vi "from string.vi"(8 "error in":errorcluster, 9 "data":string, 10 "version":string, 11 "CVT configuration in":refnum<class "CVT configuration.lvclass">) -> (0 "error out":errorcluster, 3 "CVT configuration out":refnum<class "CVT configuration.lvclass">)   [LabVIEW 2013, in "CVT configuration.lvclass"]
doc: "Provides an interface for loading a module configuration from a file or other serialized data source. It is recommended that all children of this class store data in two sets--data required for its own initialization, and any data required for parent initialization--and that each implementation uses the <b>Call Parent Method</b> primitive to de-serialize parent information. As a result, it is expected that every module configuration class calls <b>component configuration.lvclass:From String.vi</b>."
uses:
  CVT configuration.lvclass
  <vilib>/NI/Tag Bus Module Framework/channel/TBM channel.lvclass
  <vilib>/NI/Tag Bus Module Framework/module configuration/TBM module configuration.lvclass
  CVT configuration.lvclass/CVT configuration.ctl
  <vilib>/NI/Configuration Framework/serializable configuration/NISE_CEF_serializable configuration.lvclass
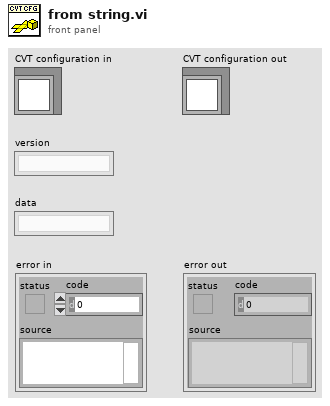
[diagram p1: front panel]
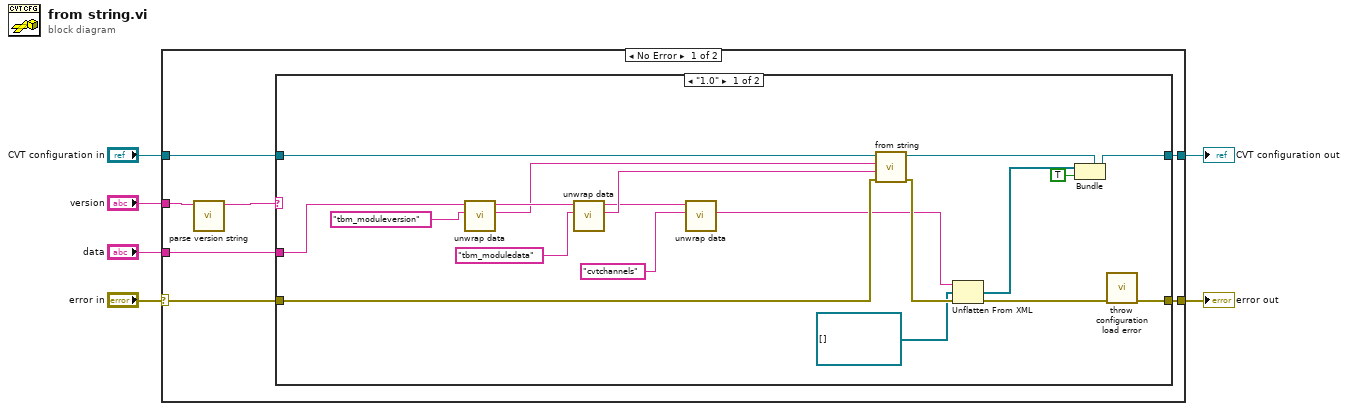
[diagram p0: block diagram]
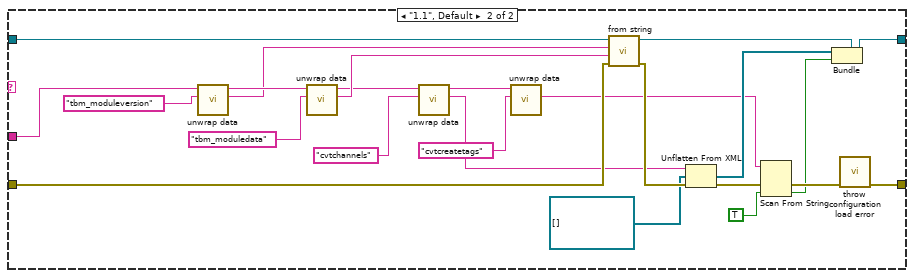
[diagram p2: hidden frame]
diagram:
  n1 = case shown="No Error" "error in" {
    selector: "error in" -> [w7 w58]
    tunnel: "data" -> [w13 _]
    tunnel: "CVT configuration in" -> [w12 w57]
    tunnel: [w11 w57] -> w5
    tunnel: [w10 w58] -> w4
    tunnel: "version" -> [w9 _]
    frame No Error {
      n2 = call <vilib>:"parse version string.vi"("full version"=w9) -> ("major.minor version"=w8:string)  [unwired: 7 in, 3 out]
      n3 = case shown="\"1.0\"" w8 {
        tunnel: w13 -> [w27 w51]
        tunnel: w7 -> [w26 w50]
        tunnel: w12 -> [w32 w56]
        tunnel: [w21 w45] -> w11
        tunnel: [w29 w53] -> w10
        frame "1.0" {
          n4 = call <vilib>:"unwrap data.vi"("identifier"="tbm_moduleversion" ("additional identifier"), "data to unwrap"=w27) -> ("unwrapped data"=w22:string, "remaining string"=w28:string)  [unwired: 8 in]
          n5 = call <vilib>:"unwrap data.vi"("identifier"="tbm_moduledata" ("additional identifier"), "data to unwrap"=w28) -> ("unwrapped data"=w24:string, "remaining string"=w17:string)  [unwired: 8 in]
          n6 = call <vilib>:"unwrap data.vi"("identifier"="cvtchannels" ("additional identifier"), "data to unwrap"=w17) -> ("unwrapped data"=w15:string)  [unwired: 8 in, 1 out]
          n7 = call-parent "from string.vi"("error in"=w26, "data"=w24, "version"=w22, "module configuration in"=w32) -> ("error out"=w30:errorcluster, "module configuration out"=w31:refnum<class "CVT configuration.lvclass">)  [unwired: 6 in]
          n8 = Unflatten From XML(xml string=w15, type=refnum<class "TBM channel.lvclass">[] [] ("channels"), error in (no error)=w30) -> (value=w18:refnum<class "TBM channel.lvclass">[], error out=w20:errorcluster)
          n9 = Bundle(cluster=w31, w18, TRUE ("Create Tags?")) -> (w21:refnum<class "CVT configuration.lvclass">)
          n10 = call <vilib>:"throw configuration load error.vi"("error in"=w20) -> ("error out"=w29:errorcluster)  [unwired: 10 in]
        }
        frame "1.1", Default {
          n11 = call <vilib>:"unwrap data.vi"("identifier"="tbm_moduleversion" ("additional identifier"), "data to unwrap"=w51) -> ("unwrapped data"=w46:string, "remaining string"=w52:string)  [unwired: 8 in]
          n12 = call <vilib>:"unwrap data.vi"("identifier"="tbm_moduledata" ("additional identifier"), "data to unwrap"=w52) -> ("unwrapped data"=w48:string, "remaining string"=w42:string)  [unwired: 8 in]
          n13 = call <vilib>:"unwrap data.vi"("identifier"="cvtchannels" ("additional identifier"), "data to unwrap"=w42) -> ("unwrapped data"=w40:string, "remaining string"=w39:string)  [unwired: 8 in]
          n14 = call <vilib>:"unwrap data.vi"("identifier"="cvtcreatetags", "data to unwrap"=w39) -> ("unwrapped data"=w35:string)  [unwired: 8 in, 1 out]
          n15 = call-parent "from string.vi"("error in"=w50, "data"=w48, "version"=w46, "module configuration in"=w56) -> ("error out"=w54:errorcluster, "module configuration out"=w55:refnum<class "CVT configuration.lvclass">)  [unwired: 6 in]
          n16 = Unflatten From XML(xml string=w40, type=refnum<class "TBM channel.lvclass">[] [] ("channels"), error in (no error)=w54) -> (value=w43:refnum<class "TBM channel.lvclass">[], error out=w37:errorcluster)
          n17 = Scan From String(input string=w35, error in=w37, default 1=TRUE) -> (error out=w34:errorcluster, output 1=w33:bool)  [unwired: 2 in, 2 out]
          n18 = Bundle(cluster=w55, w43, w33) -> (w45:refnum<class "CVT configuration.lvclass">)
          n19 = call <vilib>:"throw configuration load error.vi"("error in"=w34) -> ("error out"=w53:errorcluster)  [unwired: 10 in]
        }
      }
    }
    frame Error {
    }
  }
  "error out" <- w4
  "CVT configuration out" <- w5
